vi "Handle Messages.vi"(8 "error in (no error)":errorcluster, 9 "Message Data":variant, 10 "Message":string, 11 "Process In":refnum<class "Process.lvclass">) -> (0 "error out":errorcluster, 3 "Process Out":refnum<class "Process.lvclass">)   [LabVIEW 2020, in "Process.lvclass"]
doc: "This is the core VI handling incomming messages to the process. This VI should be overridden to add functionality to the process or override functionality implemented by a parent. Any message not handled should be sent to the parent method using the default case. \nEach state should be atomic and states should in general avoid enqueueing new messages from within this method, as there might be other messages interleaved in the queue from the outside. For cyclic iteration of an action, using a Helper Loop is recommended."
uses:
  Process.lvclass
  Process.lvclass/Process.ctl
  Error Handler Interface/Error Handler Interface.lvclass
  Public/Lifecycle/Lifecycle State.ctl
  Logging/Logging.lvclass
  C:/git/astemes-triarc-framework/source/Framework/Logging/Logging.lvclass
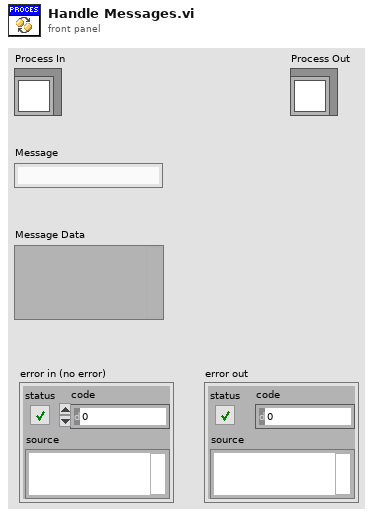
[diagram p1: front panel]
types:
  T1 = typedef "Process.lvclass/Lifecycle State.ctl" = enum16{"Uninitialized", "Initialized", "Started", "Running", "Stopped", "Finished"}
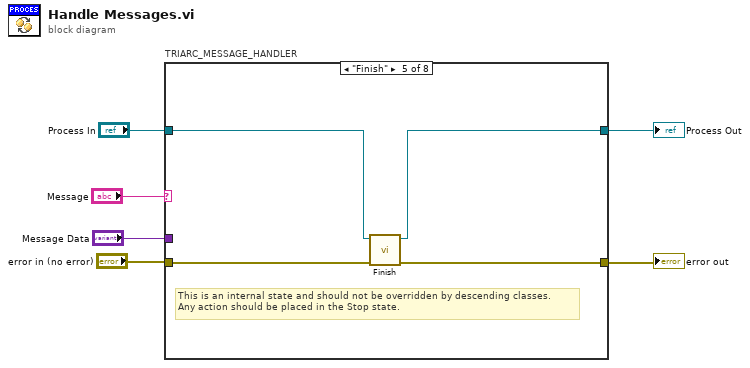
[diagram p0: block diagram]
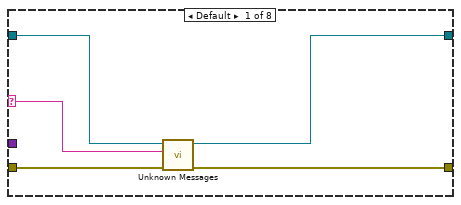
[diagram p2: hidden frame]
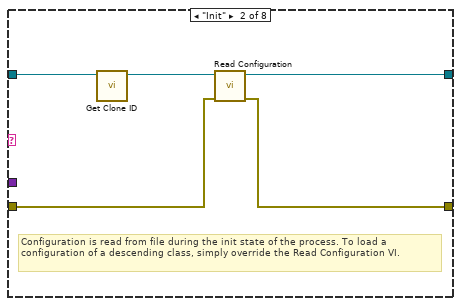
[diagram p3: hidden frame]
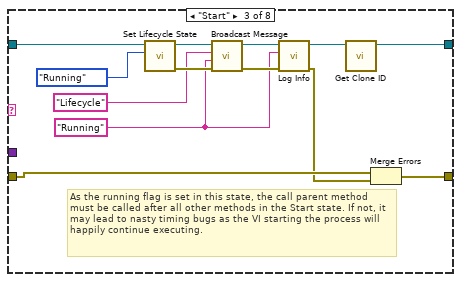
[diagram p4: hidden frame]
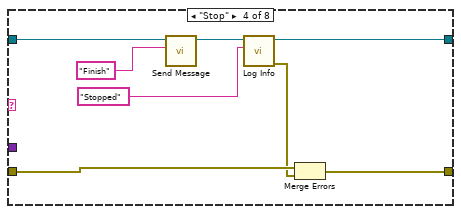
[diagram p5: hidden frame]
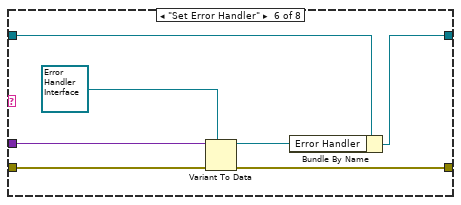
[diagram p6: hidden frame]
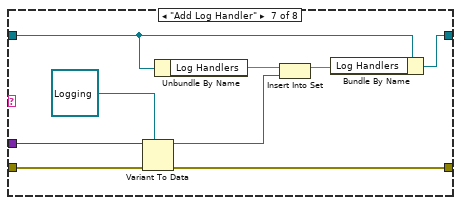
[diagram p7: hidden frame]
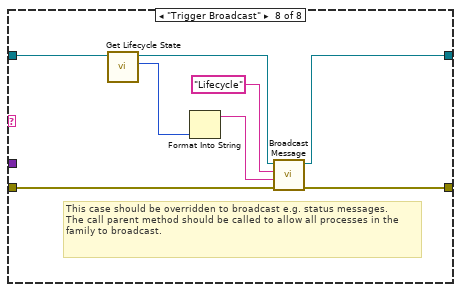
[diagram p8: hidden frame]
diagram:
  n1 = case "TRIARC_MESSAGE_HANDLER" shown="\"Finish\"" "Message" {
    selector: "Message" -> [w11 _ _ _ _ _ _ _]
    tunnel: [w8 w15 w28 w35 w41 w44 w52 w61] -> w6
    tunnel: "error in (no error)" -> [w7 w12 w27 w34 w40 w48 w57 w58]
    tunnel: [w10 w16 w18 w31 w38 w45 w54 w65] -> w4
    tunnel: "Process In" -> [w9 w13 w29 w36 w39 w46 w53 w64]
    tunnel: "Message Data" -> [_ _ _ _ _ w42 w49 _]
    frame Default {
      n2 = call "Unknown Messages.vi"("error in (no error)"=w7, "Message"=w11, "Process In"=w9) -> ("error out"=w8:errorcluster, "Process Out"=w10:refnum<class "Process.lvclass">)  [unwired: 7 in]
    }
    frame "Init" {
      # "Configuration is read from file during the init state of the process. To load a configuration of a descending class, simply override the Read Configuration VI."
      n3 = call "Get Clone ID.vi"("Process in"=w13) -> ("Process out"=w14:refnum<class "Process.lvclass">)  [unwired: 10 in]
      n4 = call-dynamic "Read Configuration.vi"("error in (no error)"=w12, "Process In"=w14) -> ("error out"=w15:errorcluster, "Process Out"=w16:refnum<class "Process.lvclass">)  [unwired: 8 in]
    }
    frame "Start" {
      w17 = "Running" ("Message")
      # "As the running flag is set in this state, the call parent method must be called after all other methods in the Start state. If not, it may lead to nasty timing bugs as the VI starting the process will happily continue executing."
      n5 = call "Set Lifecycle State.vi"("Lifecycle State"=Lifecycle_State."Running", "Process In"=w29) -> ("error out"=w25:errorcluster, "Process Out"=w26:refnum<class "Process.lvclass">)  [unwired: 8 in]
      n6 = call-dynamic "Broadcast Message.vi"("error in (no error)"=w25, "Message Data"=w17, "Message"="Lifecycle", "Process In"=w26) -> ("error out"=w24:errorcluster, "Process Out"=w21:refnum<class "Process.lvclass">)  [unwired: 6 in]
      n7 = call "Log Info.vi"("error in (no error)"=w24, "Message"=w17, "Logging In"=w21) -> ("error out"=w20:errorcluster, "Logging Out"=w19:refnum<class "Process.lvclass">)  [unwired: 7 in]
      n8 = call "Get Clone ID.vi"("Process in"=w19) -> ("Process out"=w18:refnum<class "Process.lvclass">)  [unwired: 10 in]
      n9 = Merge Errors(w27, w20) -> (w28:errorcluster)
    }
    frame "Stop" {
      n10 = call "Send Message.vi"("Message"="Finish", "Process In"=w36) -> ("Process Out"=w32:refnum<class "Process.lvclass">)  [unwired: 8 in, 1 out]
      n11 = call "Log Info.vi"("Message"="Stopped", "Logging In"=w32) -> ("error out"=w33:errorcluster, "Logging Out"=w31:refnum<class "Process.lvclass">)  [unwired: 8 in]
      n12 = Merge Errors(w34, w33) -> (w35:errorcluster)
    }
    frame "Finish" {
      # "This is an internal state and should not be overridden by descending classes.\nAny action should be placed in the Stop state."
      n13 = call "Finish.vi"("error in (no error)"=w40, "Process In"=w39) -> ("error out"=w41:errorcluster, "Process Out"=w38:refnum<class "Process.lvclass">)  [unwired: 8 in]
    }
    frame "Set Error Handler" {
      n14 = Variant To Data(error in=w48, type=refnum<class "Error Handler Interface.lvclass"> refnum ("Error Handler Interface.lvclass"), Variant=w42) -> (data=w43:refnum<class "Error Handler Interface.lvclass">, error out=w44:errorcluster)
      n15 = Bundle By Name(cluster=w46, "Error Handler"=w43) -> (w45:refnum<class "Process.lvclass">)
    }
    frame "Add Log Handler" {
      n16 = Variant To Data(error in=w57, type=refnum<class "Logging.lvclass"> refnum ("element"), Variant=w49) -> (data=w50:refnum<class "Logging.lvclass">, error out=w52:errorcluster)
      n17 = Unbundle By Name(w53) -> ("Log Handlers"=w55:set{refnum<class "Logging.lvclass">})
      n18 = Insert Into Set(10:w50, 11:w55) -> (3:w56:set{refnum<class "Logging.lvclass">})  [unwired: 1 out]
      n19 = Bundle By Name(cluster=w53, "Log Handlers"=w56) -> (w54:refnum<class "Process.lvclass">)
    }
    frame "Trigger Broadcast" {
      # "This case should be overridden to broadcast e.g. status messages.\nThe call parent method should be called to allow all processes in the family to broadcast."
      n20 = call "Get Lifecycle State.vi"("Process In"=w64) -> ("Lifecycle State"=w60:T1, "Process Out"=w62:refnum<class "Process.lvclass">)  [unwired: 7 in, 2 out]
      n21 = Format Into String(w60) -> (resulting string=w59:string)  [unwired: 3 in, 1 out]
      n22 = call-dynamic "Broadcast Message.vi"("error in (no error)"=w58, "Message Data"=w59, "Message"="Lifecycle", "Process In"=w62) -> ("error out"=w61:errorcluster, "Process Out"=w65:refnum<class "Process.lvclass">)  [unwired: 6 in]
    }
  }
  "error out" <- w6
  "Process Out" <- w4
